vi "test Parsed XML to System Definition.vi"(8 "error in":errorcluster, 11 "TestCase in":refnum<class "Scripting.lvclass">) -> (0 "error out":errorcluster, 3 "TestCase out":refnum<class "Scripting.lvclass">)   [LabVIEW 2020, in "Scripting.lvclass"]
uses:
  Scripting.lvclass
  Scripting.lvclass/Scripting.ctl
  C:/Program Files/National Instruments/LabVIEW 2026/vi.lib/addons/_JKI Toolkits/VI Tester/TestCase.llb/TestCase.lvclass
  C:/git/fmussi_niveristand-aim-arinc429-custom-device/Source/Custom Device Support/Tests/Unit/Scripting/Scripting.lvclass
  <vilib>/addons/_JKI Toolkits/VI Tester/TestCase.llb/TestCase.lvclass
  Scripting/AIM/AIM ARINC 429 Scripting.lvlib
  <userlib>/_OpenG.lib/appcontrol/appcontrol.llb/openg_application_control.lvlib
  <vilib>/NI/VeriStand Custom Device Testing Tools/VeriStandTestUtilities/VeriStandTestUtilities.lvlib
  Shared/VS Channels Definition for Label.ctl
  Shared/VS Channels Definition for All Labels on Hardware Channel.ctl
  <vilib>/NI/NI VeriStand Encoding and Decoding/Encoding.ctl
  <vilib>/NI/NI VeriStand Encoding and Decoding/Encoding and Decoding.lvlib
  Shared/Parameter Definition.ctl
  Shared/VS Channel Definition for Parameter.ctl
  Shared/Direction.ctl
  Shared/Transfer Type.ctl
  Shared/Transfer Speed.ctl
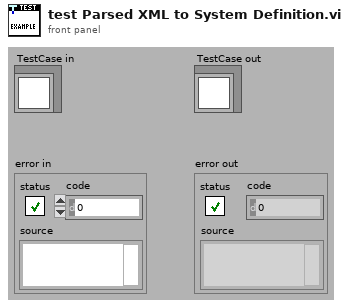
[diagram p1: front panel]
types:
  T1 = typedef "VS Channels Definition for All Labels on Hardware Channel.ctl" = cluster{"hardware channel":i32, "direction":T2, "labels":T3[], "speed":T8}
  T2 = typedef "Direction.ctl" = enum16{"Rx", "Tx"}
  T3 = typedef "VS Channels Definition for Label.ctl" = cluster{"label (Dec)":u32, "parameters":T4[], "SDI value":u8, "SDI enabled":bool, "transfer type":T7, "create timestamp":bool, "transmit period":u32}
  T4 = typedef "VS Channel Definition for Parameter.ctl" = cluster{"name":string, "unit":string, "Parameter":T5}
  T5 = typedef "Parameter Definition.ctl" = cluster{"start index":i32, "size":i32, "encoding":T6, "signed":bool, "scale multiplier":dbl, "scale offset":dbl, "default value":dbl}
  T6 = typedef "Encoding and Decoding.lvlib/Encoding.ctl" = enum16{"BNR", "BCD", "Discrete"}
  T7 = typedef "Transfer Type.ctl" = enum16{"Scheduled", "Acyclic", "Block", "Strobe"}
  T8 = typedef "Transfer Speed.ctl" = enum16{"LO (12.5 kb/s)", "HI (100 kb/s)"}
  T9 = typedef "Custom Device API.lvlib/Custom Device Item Ref.ctl" = u64
  T10 = typedef "Label Properties.ctl" = cluster{"label (Dec)":T11, "SDI value":u8, "SDI enabled":bool}
  T11 = typedef "Label.ctl" = u8
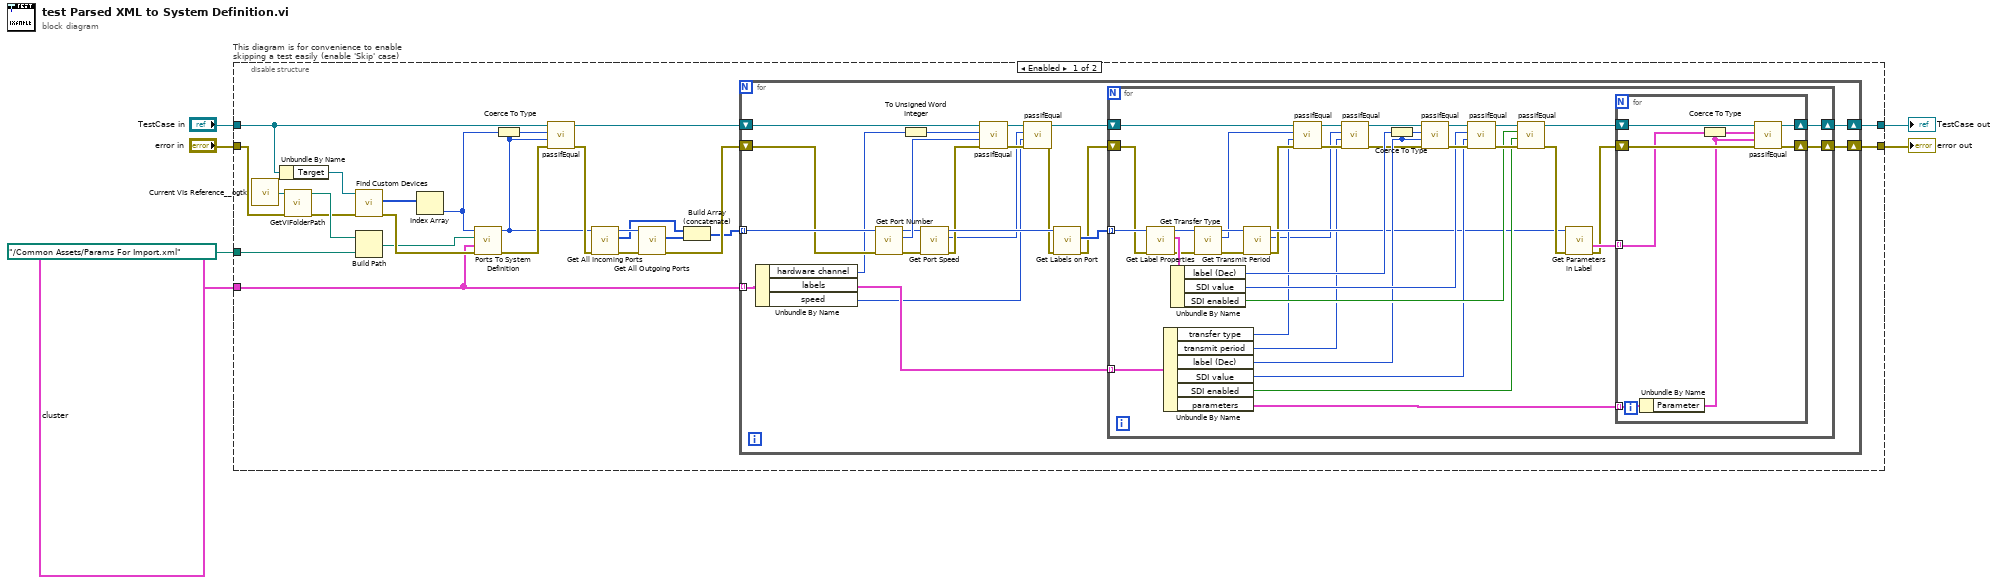
[diagram p0: block diagram]
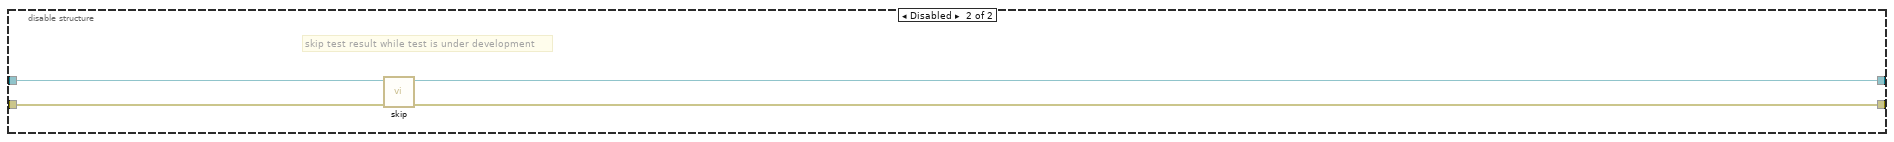
[diagram p2: hidden frame]
diagram:
  n1 = disable-structure "This diagram is for convenience to enable skipping a test easily (enable 'Skip' case)" shown="Enabled" {
    disable-tunnel: "TestCase in" -> [w24 w102]
    disable-tunnel: [w14 w100] -> w3
    disable-tunnel: [w12 w101] -> w5
    disable-tunnel: "error in" -> [w27 w99]
    disable-tunnel: T1[] [{"hardware channel"=0, "direction"=enum."Rx", "labels"=[{"label (Dec)"=134, "parameters"=[{"name"="Altitude_Rx", "unit"="psi", "Parameter"={"start index"=18, "size"=10, "encoding"=enum."BNR", "signed"=TRUE, "scale multiplier"=16.0, "scale offset"=0.0, "default value"=0.0}}, {"name"="SSM", "unit"="", "Parameter"={"start index"=29, "size"=2, "encoding"=enum."BNR", "signed"=FALSE, "scale multiplier"=1.0, "scale offset"=0.0, "default value"=0.0}}], "SDI value"=0, "SDI enabled"=FALSE, "transfer type"=enum."Scheduled", "create timestamp"=FALSE, "transmit period"=1000}], "speed"=enum."LO (12.5 kb/s)"}, {"hardware channel"=2, "direction"=enum."Rx", "labels"=[{"label (Dec)"=135, "parameters"=[{"name"="Altitude_Rx", "unit"="ft", "Parameter"={"start index"=10, "size"=19, "encoding"=enum."BCD", "signed"=TRUE, "scale multiplier"=1.0, "scale offset"=0.0, "default value"=0.0}}, {"name"="SSM", "unit"="", "Parameter"={"start index"=29, "size"=2, "encoding"=enum."BNR", "signed"=FALSE, "scale multiplier"=1.0, "scale offset"=0.0, "default value"=0.0}}], "SDI value"=2, "SDI enabled"=TRUE, "transfer type"=enum."Scheduled", "create timestamp"=FALSE, "transmit period"=1000}], "speed"=enum."HI (100 kb/s)"}, {"hardware channel"=4, "direction"=enum."Rx", "labels"=[{"label (Dec)"=136, "parameters"=[{"name"="Altitude_Rx", "unit"="m", "Parameter"={"start index"=13, "size"=16, "encoding"=enum."BNR", "signed"=TRUE, "scale multiplier"=1.0, "scale offset"=0.0, "default value"=0.0}}, {"name"="valid_Rx", "unit"="", "Parameter"={"start index"=10, "size"=1, "encoding"=enum."Discrete", "signed"=FALSE, "scale multiplier"=1.0, "scale offset"=0.0, "default value"=0.0}}, {"name"="current_Rx", "unit"="", "Parameter"={"start index"=11, "size"=1, "encoding"=enum."Discrete", "signed"=FALSE, "scale multiplier"=1.0, "scale offset"=0.0, "default value"=0.0}}, {"name"="SSM", "unit"="", "Parameter"={"start index"=29, "size"=2, "encoding"=enum."BNR", "signed"=FALSE, "scale multiplier"=1.0, "scale offset"=0.0, "default value"=0.0}}], "SDI value"=0, "SDI enabled"=FALSE, "transfer type"=enum."Scheduled", "create timestamp"=FALSE, "transmit period"=1000}], "speed"=enum."HI (100 kb/s)"}, {"hardware channel"=17, "direction"=enum."Tx", "labels"=[{"label (Dec)"=134, "parameters"=[{"name"="Altitude_Tx", "unit"="psi", "Parameter"={"start index"=18, "size"=10, "encoding"=enum."BNR", "signed"=TRUE, "scale multiplier"=16.0, "scale offset"=0.0, "default value"=0.0}}], "SDI value"=0, "SDI enabled"=FALSE, "transfer type"=enum."Scheduled", "create timestamp"=FALSE, "transmit period"=20000}], "speed"=enum."HI (100 kb/s)"}, {"hardware channel"=19, "direction"=enum."Tx", "labels"=[{"label (Dec)"=135, "parameters"=[{"name"="Altitude_Tx", "unit"="ft", "Parameter"={"start index"=10, "size"=19, "encoding"=enum."BCD", "signed"=TRUE, "scale multiplier"=1.0, "scale offset"=0.0, "default value"=0.0}}], "SDI value"=2, "SDI enabled"=TRUE, "transfer type"=enum."Scheduled", "create timestamp"=FALSE, "transmit period"=50000}], "speed"=enum."HI (100 kb/s)"}, {"hardware channel"=21, "direction"=enum."Tx", "labels"=[{"label (Dec)"=136, "parameters"=[{"name"="Altitude_Tx", "unit"="m", "Parameter"={"start index"=13, "size"=16, "encoding"=enum."BNR", "signed"=TRUE, "scale multiplier"=1.0, "scale offset"=0.0, "default value"=0.0}}, {"name"="valid_Tx", "unit"="", "Parameter"={"start index"=10, "size"=1, "encoding"=enum."Discrete", "signed"=FALSE, "scale multiplier"=1.0, "scale offset"=0.0, "default value"=0.0}}, {"name"="current_Tx", "unit"="", "Parameter"={"start index"=11, "size"=1, "encoding"=enum."Discrete", "signed"=FALSE, "scale multiplier"=1.0, "scale offset"=0.0, "default value"=0.0}}], "SDI value"=0, "SDI enabled"=FALSE, "transfer type"=enum."Acyclic", "create timestamp"=FALSE, "transmit period"=1000}], "speed"=enum."LO (12.5 kb/s)"}] ("ports") -> [w8 _]
    disable-tunnel: path "../Common Assets/Params For Import.xml" ("Absolute or Relative Path") -> [w25 _]
    frame Enabled {
      n2 = call <userlib>:"Current VIs Reference__ogtk.vi"() -> ("Current VI's reference"=w28:refnum<vi>)  [unwired: 5 in]
      n3 = Unbundle By Name(w24) -> ("Target"=w31:refnum<k24>)
      n4 = call <vilib>:"GetVIFolderPath.vi"("error in (no error)"=w27, "VI Reference in"=w28) -> ("error out"=w26:errorcluster, "VI Folder Path out"=w29:path)  [unwired: 8 in]
      n5 = call "Find Custom Devices.vi"("error in"=w26, "target"=w31) -> ("error out"=w30:errorcluster, "AIM ARINC 429 custom devices"=w7:T9[])  [unwired: 7 in, 1 out]
      n6 = Build Path(base path=w29, name or relative path=w25) -> (appended path=w9:path)
      n7 = Index Array(array=w7) -> (element=w22:T9)  [unwired: 1 in]
      n8 = call "Ports To System Definition.vi"("error in"=w30, "ports"=w8, "parameter configuration file path"=w9, "custom device ref"=w22) -> ("error out"=w23:errorcluster, "custom device ref out"=w10:T9)  [unwired: 6 in]
      n9 = Coerce To Type(0:w22, 1:w10) -> (2:w11:T9)
      n10 = call-dynamic "passIfEqual.vi"("error in (no error)"=w23, "y"=w10, "x"=w11, "TestCase in"=w24) -> ("error out"=w21:errorcluster, "TestCase out"=w13:refnum<class "Scripting.lvclass">)  [unwired: 6 in]
      n11 = call "Get All Incoming Ports.vi"("error in"=w21, "custom device ref"=w10) -> ("error out"=w19:errorcluster, "incoming ports"=w16:T9[], "custom device ref out"=w20:T9)  [unwired: 7 in]
      n12 = call "Get All Outgoing Ports.vi"("error in"=w19, "custom device ref"=w20) -> ("error out"=w18:errorcluster, "outgoing ports"=w17:T9[])  [unwired: 7 in, 1 out]
      n13 = Build Array (concatenate)(w16, w17) -> (w15:T9[])
      n14 = for {
        tunnel: w15 -> [w52] mode=indexing
        tunnel: w8 -> [w53] mode=indexing
        shift-right: [w50] -> w12
        shift-left: w18 -> [w51]
        shift-right: [w44] -> w14
        shift-left: w13 -> [w47]
        n15 = Unbundle By Name(w53) -> ("hardware channel"=w46:i32, "labels"=w48:T3[], "speed"=w32:T8)
        n16 = call "Get Port Number.vi"("error in"=w51, "port ref"=w52) -> ("error out"=w42:errorcluster, "port number"=w45:u16, "port ref out"=w41:T9)  [unwired: 6 in, 1 out]
        n17 = To Unsigned Word Integer(number=w46) -> (unsigned 16bit integer=w43:u16)
        n18 = call "Get Port Speed.vi"("error in"=w42, "port ref"=w41) -> ("error out"=w36:errorcluster, "speed"=w33:T8, "port ref out"=w37:T9)  [unwired: 7 in]
        n19 = call-dynamic "passIfEqual.vi"("error in (no error)"=w36, "y"=w45, "x"=w43, "TestCase in"=w47) -> ("error out"=w40:errorcluster, "TestCase out"=w39:refnum<class "Scripting.lvclass">)  [unwired: 6 in]
        n20 = call-dynamic "passIfEqual.vi"("error in (no error)"=w40, "y"=w32, "x"=w33, "TestCase in"=w39) -> ("error out"=w35:errorcluster, "TestCase out"=w38:refnum<class "Scripting.lvclass">)  [unwired: 6 in]
        n21 = call "Get Labels on Port.vi"("error in"=w35, "port ref"=w37) -> ("error out"=w34:errorcluster, "labels"=w49:T9[])  [unwired: 6 in, 2 out]
        n22 = for {
          shift-right: [w77] -> w50
          shift-left: w34 -> [w89]
          tunnel: w49 -> [w90] mode=indexing
          tunnel: w48 -> [w88] mode=indexing
          shift-right: [w78] -> w44
          shift-left: w38 -> [w63]
          n23 = call "Get Label Properties.vi"("error in"=w89, "label ref"=w90) -> ("error out"=w69:errorcluster, "label properties"=w87:T10, "label ref out"=w70:T9)  [unwired: 6 in, 1 out]
          n24 = Unbundle By Name(w88) -> ("transfer type"=w56:T7, "transmit period"=w54:u32, "label (Dec)"=w73:u32, "SDI value"=w74:u8, "SDI enabled"=w75:bool, "parameters"=w85:T4[])
          n25 = Unbundle By Name(w87) -> ("label (Dec)"=w72:T11, "SDI value"=w80:u8, "SDI enabled"=w76:bool)
          n26 = call "Get Transfer Type.vi"("error in"=w69, "label ref"=w70) -> ("error out"=w66:errorcluster, "transfer type"=w61:T7, "label ref out"=w65:T9)  [unwired: 7 in]
          n27 = call "Get Transmit Period.vi"("error in"=w66, "label ref"=w65) -> ("error out"=w62:errorcluster, "transmit period (us)"=w55:u32, "label ref out"=w64:T9)  [unwired: 7 in]
          n28 = call-dynamic "passIfEqual.vi"("error in (no error)"=w62, "y"=w56, "x"=w61, "TestCase in"=w63) -> ("error out"=w60:errorcluster, "TestCase out"=w59:refnum<class "Scripting.lvclass">)  [unwired: 6 in]
          n29 = call-dynamic "passIfEqual.vi"("error in (no error)"=w60, "y"=w54, "x"=w55, "TestCase in"=w59) -> ("error out"=w58:errorcluster, "TestCase out"=w57:refnum<class "Scripting.lvclass">)  [unwired: 6 in]
          n30 = Coerce To Type(0:w72, 1:w73) -> (2:w71:u32)
          n31 = call-dynamic "passIfEqual.vi"("error in (no error)"=w58, "y"=w73, "x"=w71, "TestCase in"=w57) -> ("error out"=w81:errorcluster, "TestCase out"=w82:refnum<class "Scripting.lvclass">)  [unwired: 6 in]
          n32 = call-dynamic "passIfEqual.vi"("error in (no error)"=w81, "y"=w74, "x"=w80, "TestCase in"=w82) -> ("error out"=w84:errorcluster, "TestCase out"=w83:refnum<class "Scripting.lvclass">)  [unwired: 6 in]
          n33 = call-dynamic "passIfEqual.vi"("error in (no error)"=w84, "y"=w75, "x"=w76, "TestCase in"=w83) -> ("error out"=w68:errorcluster, "TestCase out"=w79:refnum<class "Scripting.lvclass">)  [unwired: 6 in]
          n34 = call "Get Parameters in Label.vi"("error in"=w68, "label ref"=w64) -> ("error out"=w67:errorcluster, "parameter definitions"=w86:T5[])  [unwired: 6 in, 2 out]
          n35 = for {
            tunnel: w86 -> [w95] mode=indexing
            tunnel: w85 -> [w98] mode=indexing
            shift-right: [w93] -> w78
            shift-left: w79 -> [w97]
            shift-right: [w94] -> w77
            shift-left: w67 -> [w96]
            n36 = Unbundle By Name(w98) -> ("Parameter"=w91:T5)
            n37 = Coerce To Type(0:w95, 1:w91) -> (2:w92:T5)
            n38 = call-dynamic "passIfEqual.vi"("error in (no error)"=w96, "y"=w91, "x"=w92, "TestCase in"=w97) -> ("error out"=w94:errorcluster, "TestCase out"=w93:refnum<class "Scripting.lvclass">)  [unwired: 6 in]
          }
        }
      }
    }
    frame Disabled {
      # "skip test result while test is under development"
      n39 = call <vilib>:"skip.vi"("error in (no error)"=w99, "TestCase in"=w102) -> ("error out"=w101:errorcluster, "TestCase out"=w100:refnum<class "Scripting.lvclass">)  [unwired: 8 in]
    }
  }
  "error out" <- w5
  "TestCase out" <- w3
